vi "DTCs.Codes.Get.vi"(8 "error in (no error)":errorcluster, 10 "Addon Name":string, 11 "Address":string) -> (0 "error out":errorcluster, 3 "Codes":T1)   [LabVIEW 2025, in "Diagnostics Addon Shared.lvlib"]
uses:
  Diagnostics Addon Shared.lvlib
  Types/DTC.Codes.ctl
  Constants.vi
  NationalInstruments.VeriStand.SystemDefinitionAPI
  NationalInstruments.VeriStand.SystemStorage
  <vilib>/NI VeriStand/Execution/Workspace/NI_VS Workspace ExecutionAPI.lvlib
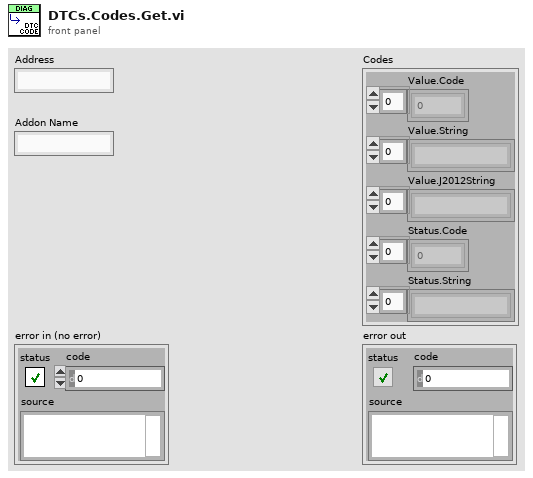
[diagram p1: front panel]
types:
  T1 = typedef "Diagnostics Addon Shared.lvlib/DTC.Codes.ctl" = cluster{"Value.Code":dbl[], "Value.String":string[], "Value.J2012String":string[], "Status.Code":dbl[], "Status.String":string[]}
  T2 = typedef "NI_VS Workspace ExecutionAPI.lvlib/WorkspaceAPI.ctl" = refnum<k24>
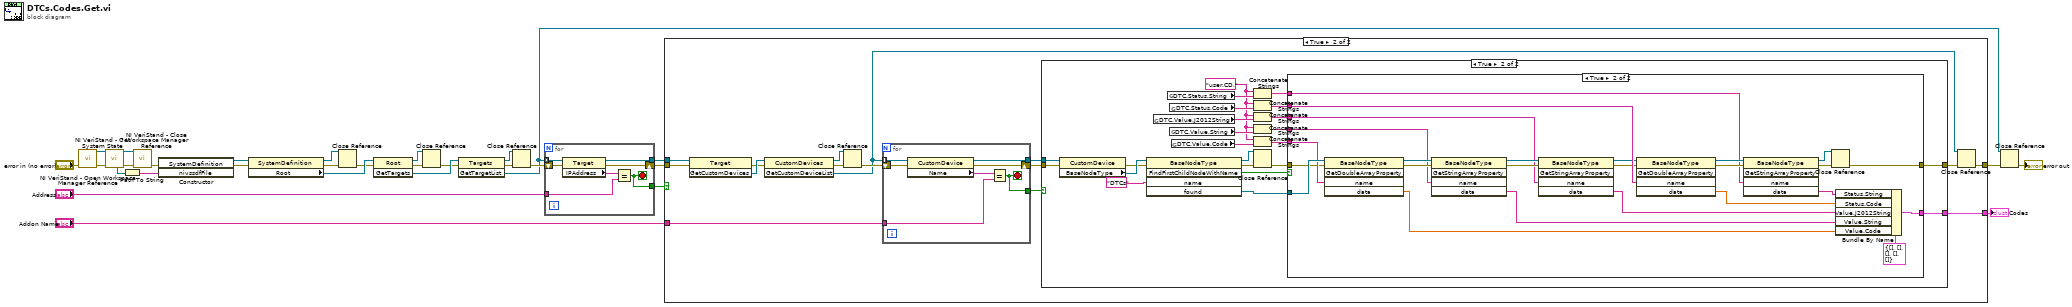
[diagram p0: block diagram]
diagram:
  n1 = call <vilib>:"NI VeriStand - Open Workspace Manager Reference.vi"("error in (no error)"="error in (no error)") -> ("error out"=w30:errorcluster, "WorkspaceManager"=w29:T2)  [unwired: 9 in]
  n2 = call <vilib>:"NI VeriStand - Get System State.vi"("error in (no error)"=w30, "WorkspaceManager in"=w29) -> ("error out"=w28:errorcluster, "WorkspaceManager  out"=w27:T2, "System Definition File"=w26:path)  [unwired: 5 in, 2 out]
  n3 = Path To String(path=w26) -> (string=w25:string)
  n4 = call <vilib>:"NI VeriStand - Close Workspace Manager Reference.vi"("error in (no error)"=w28, "WorkspaceManager"=w27) -> ("error out"=w24:errorcluster)  [unwired: 9 in]
  n5 = constructor class="SystemDefinition"(error in=w24, "nivssdfFile"=w25) -> (reference out=w23:refnum<k24>, error out=w22:errorcluster)  [unwired: 2 in, 2 out]
  n6 = property class="SystemDefinition"(reference=w23, error in=w22) -> (reference out=w17:refnum<k24>, error out=w16:errorcluster, "Root"=w21:refnum<k24>)
  n7 = Close Reference(reference=w17, error in (no error)=w16) -> (error out=w15:errorcluster)
  n8 = invoke class="Root" method="GetTargets"(reference=w21, error in=w15) -> (reference out=w12:refnum<k24>, error out=w14:errorcluster, "GetTargets"=w20:refnum<k24>)  [unwired: 1 in]
  n9 = Close Reference(reference=w12, error in (no error)=w14) -> (error out=w13:errorcluster)
  n10 = invoke class="Targets" method="GetTargetList"(reference=w20, error in=w13) -> (reference out=w9:refnum<k24>, error out=w11:errorcluster, "GetTargetList"=w6:refnum<k24>[])  [unwired: 1 in]
  n11 = Close Reference(reference=w9, error in (no error)=w11) -> (error out=w10:errorcluster)
  n12 = for {
    tunnel: w6 -> [w37] mode=indexing
    shift-right: [w35] -> w8
    shift-left: w10 -> [w36]
    tunnel: "Address" -> [w33]
    tunnel: [w32] -> w19
    tunnel: [w31] -> w18
    stop <- w32 stop-if-true
    n13 = property class="Target"(reference=w37, error in=w36) -> (reference out=w31:refnum<k24>, error out=w35:errorcluster, "IPAddress"=w34:string)
    n14 = Equal?(x=w34, y=w33) -> (x = y?=w32:bool)
  }
  n15 = case shown="True" w19 {
    tunnel: w18 -> [_ w53]
    tunnel: w8 -> [w38 w52]
    tunnel: "Addon Name" -> [_ w49]
    tunnel: [w38 w40] -> w7
    tunnel: [_ w39] -> w4
    frame False {
    }
    frame True {
      n16 = invoke class="Target" method="GetCustomDevices"(reference=w53, error in=w52) -> (error out=w50:errorcluster, "GetCustomDevices"=w51:refnum<k24>)  [unwired: 1 in, 1 out]
      n17 = invoke class="CustomDevices" method="GetCustomDeviceList"(reference=w51, error in=w50) -> (reference out=w43:refnum<k24>, error out=w45:errorcluster, "GetCustomDeviceList"=w41:refnum<k24>[])  [unwired: 1 in]
      n18 = Close Reference(reference=w43, error in (no error)=w45) -> (error out=w44:errorcluster)
      n19 = for {
        tunnel: w41 -> [w110] mode=indexing
        shift-right: [w108] -> w46
        shift-left: w44 -> [w109]
        tunnel: w49 -> [w106]
        tunnel: [w105] -> w48
        tunnel: [w104] -> w47
        stop <- w105 stop-if-true
        n20 = property class="CustomDevice"(reference=w110, error in=w109) -> (reference out=w104:refnum<k24>, error out=w108:errorcluster, "Name"=w107:string)
        n21 = Equal?(x=w107, y=w106) -> (x = y?=w105:bool)
      }
      n22 = case shown="True" w48 {
        tunnel: w47 -> [_ w77]
        tunnel: w46 -> [w54 w76]
        tunnel: [w54 w60] -> w42
        tunnel: [_ w59] -> w39
        frame False {
        }
        frame True {
          w57 = "user.CD."
          n23 = property class="CustomDevice"(reference=w77, error in=w76) -> (error out=w74:errorcluster, "BaseNodeType"=w75:refnum<k24>)  [unwired: 1 out]
          n24 = invoke class="BaseNodeType" method="FindFirstChildNodeWithName"(reference=w75, error in=w74, "name"="DTCs") -> (reference out=w63:refnum<k24>, error out=w62:errorcluster, "FindFirstChildNodeWithName"=w55:bool, "found"=w72:refnum<k24>)  [unwired: 2 in, 1 out]
          n25 = global read "Constants.vi" "DTC.Value.J2012String"() -> (w58:string)
          n26 = global read "Constants.vi" "DTC.Status.String"() -> (w68:string)
          n27 = global read "Constants.vi" "DTC.Value.String"() -> (w70:string)
          n28 = global read "Constants.vi" "DTC.Status.Code"() -> (w69:string)
          n29 = global read "Constants.vi" "DTC.Value.Code"() -> (w71:string)
          n30 = Concatenate Strings(w57, w68) -> (w64:string)
          n31 = Concatenate Strings(w57, w69) -> (w65:string)
          n32 = Concatenate Strings(w57, w58) -> (w56:string)
          n33 = Concatenate Strings(w57, w70) -> (w66:string)
          n34 = Concatenate Strings(w57, w71) -> (w67:string)
          n35 = Close Reference(reference=w63, error in (no error)=w62) -> (error out=w61:errorcluster)
          n36 = case shown="True" w55 {
            tunnel: w72 -> [_ w103]
            tunnel: w67 -> [_ w98]
            tunnel: w66 -> [_ w97]
            tunnel: w65 -> [_ w96]
            tunnel: w64 -> [_ w95]
            tunnel: w61 -> [w78 w94]
            tunnel: [w78 w91] -> w60
            tunnel: [_ w85] -> w59
            tunnel: w56 -> [_ w80]
            frame False {
            }
            frame True {
              n37 = invoke class="BaseNodeType" method="GetDoubleArrayProperty"(reference=w103, error in=w94, "name"=w98) -> (reference out=w101:refnum<k24>, error out=w102:errorcluster, "data"=w89:dbl[])  [unwired: 2 in, 2 out]
              n38 = invoke class="BaseNodeType" method="GetStringArrayProperty"(reference=w101, error in=w102, "name"=w97) -> (reference out=w83:refnum<k24>, error out=w84:errorcluster, "data"=w88:string[])  [unwired: 2 in, 2 out]
              n39 = invoke class="BaseNodeType" method="GetStringArrayProperty"(reference=w83, error in=w84, "name"=w80) -> (reference out=w82:refnum<k24>, error out=w81:errorcluster, "data"=w79:string[])  [unwired: 2 in, 2 out]
              n40 = invoke class="BaseNodeType" method="GetDoubleArrayProperty"(reference=w82, error in=w81, "name"=w96) -> (reference out=w100:refnum<k24>, error out=w99:errorcluster, "data"=w87:dbl[])  [unwired: 2 in, 2 out]
              n41 = invoke class="BaseNodeType" method="GetStringArrayProperty"(reference=w100, error in=w99, "name"=w95) -> (reference out=w92:refnum<k24>, error out=w93:errorcluster, "data"=w86:string[])  [unwired: 2 in, 2 out]
              n42 = Close Reference(reference=w92, error in (no error)=w93) -> (error out=w91:errorcluster)
              n43 = Bundle By Name(cluster=T1 {"Value.Code"=[], "Value.String"=[], "Value.J2012String"=[], "Status.Code"=[], "Status.String"=[]}, "Status.String"=w86, "Status.Code"=w87, "Value.J2012String"=w79, "Value.String"=w88, "Value.Code"=w89) -> (w85:T1)
            }
          }
        }
      }
      n44 = Close Reference(reference=w41, error in (no error)=w42) -> (error out=w40:errorcluster)
    }
  }
  "Codes" <- w4
  n45 = Close Reference(reference=w6, error in (no error)=w7) -> (error out=→"error out":errorcluster)
